vi "lvmcp_removeframe.vi"() -> ()   [LabVIEW 2015]
panel:
  out "error out":errorcluster
  in  "Frame Index":i32
  in  "reference":refnum<vi>
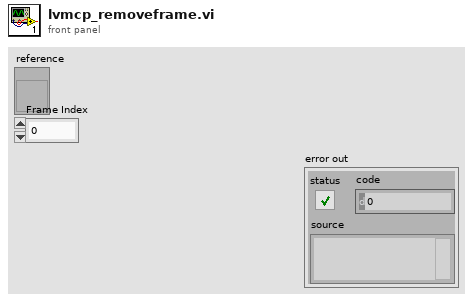
[diagram p1: front panel]
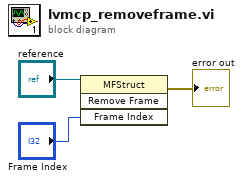
[diagram p0: block diagram]
diagram:
  n1 = invoke class="MFStruct" method="Remove Frame"(reference="reference", "Frame Index"="Frame Index") -> (error out=→"error out":errorcluster)  [unwired: 2 in, 3 out]
